vi "HI-POT_Driver.vi"(0 "VISA resource name":refnum<visa-resource-name>, 1 "?":T1, 5 "error in (no error)":errorcluster, 6 "configuration file path":path) -> (9 "Measured Voltage":string, 10 "INTERLOCK STATUS":bool, 11 "Error":bool, 12 "Current":string, 13 "Voltage":string, 14 "VISA resource name out":refnum<visa-resource-name>, 15 "Result":string, 16 "LO SET":string, 17 "Result":bool, 18 "HI SET":string, 19 "error out":errorcluster)   [LabVIEW 2021]
uses:
  Hi-pot_Driver.ctl
  GPT-9800_GSB_L8.5/GPT-9000.lvlib
panel:
  out "substring":string
  out "concatenated string":string
  out "Test Time(S)":dbl
  out "VISA resource name out 4":refnum<visa-resource-name>
  out "VISA resource name out 3":refnum<visa-resource-name>
  out "VISA resource name out 2":refnum<visa-resource-name>
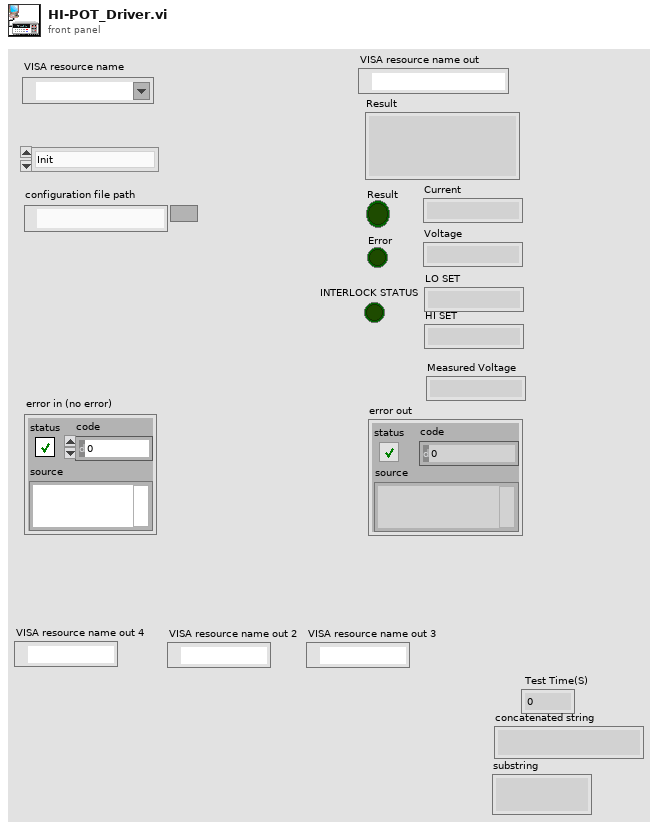
[diagram p1: front panel]
types:
  T1 = typedef "Hi-pot_Driver.ctl" = enum16{"Init ", "Interlock status", "Set UP DCW", "Set UP ACW", "Set UP IR", "Read", "Clear", "Close"}
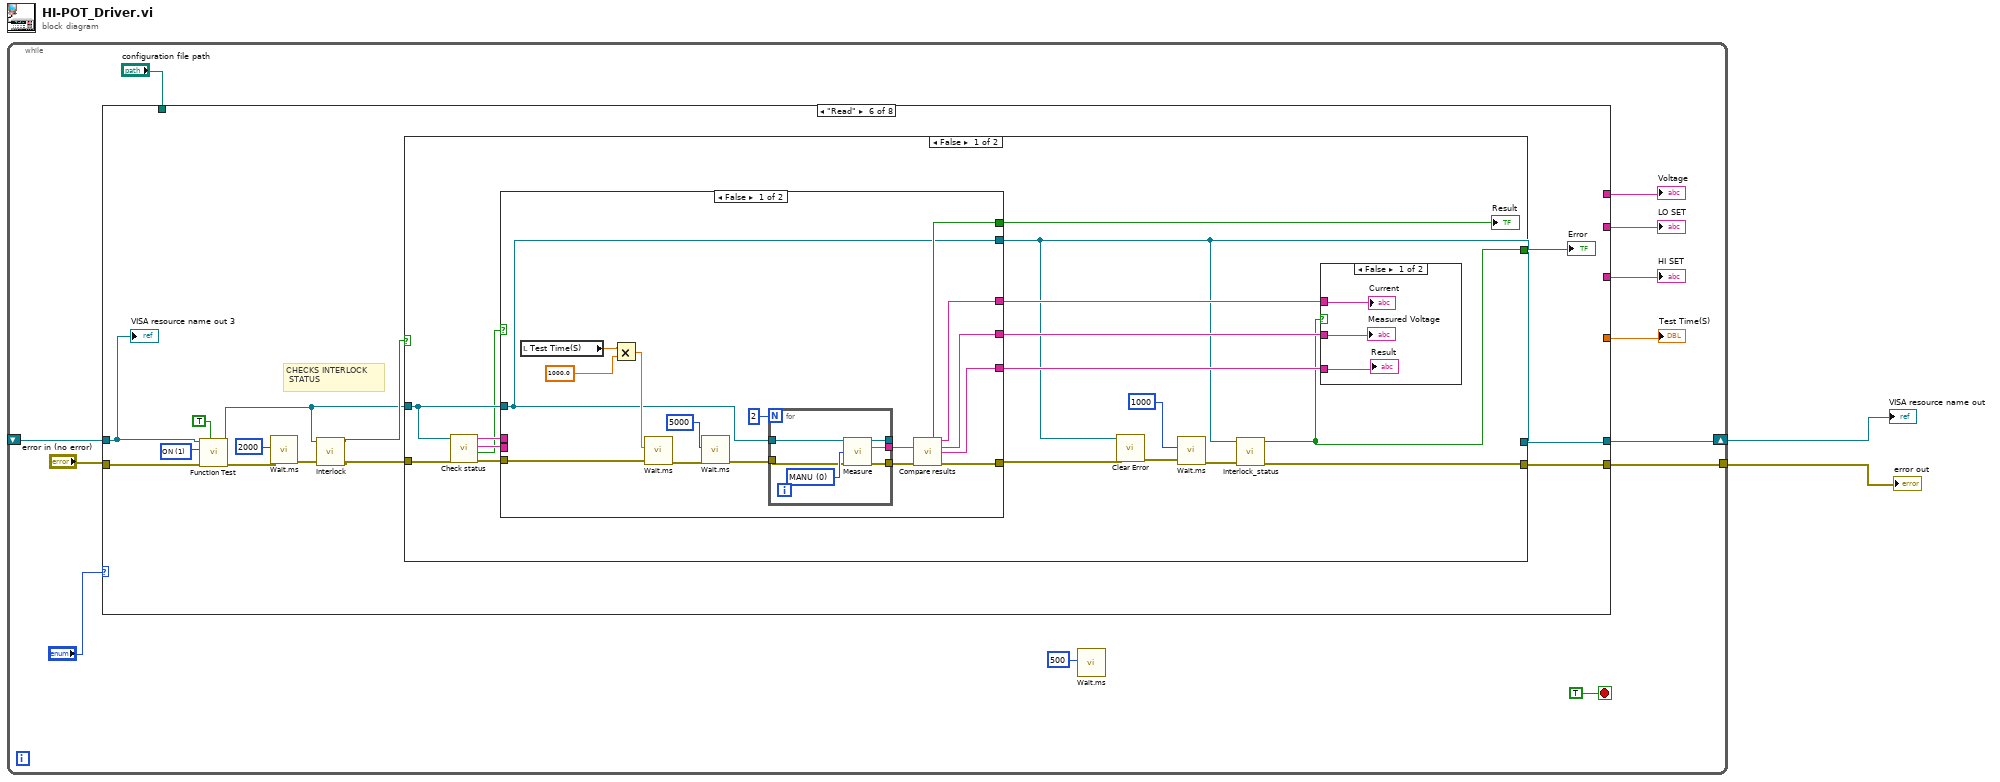
[diagram p0: block diagram]
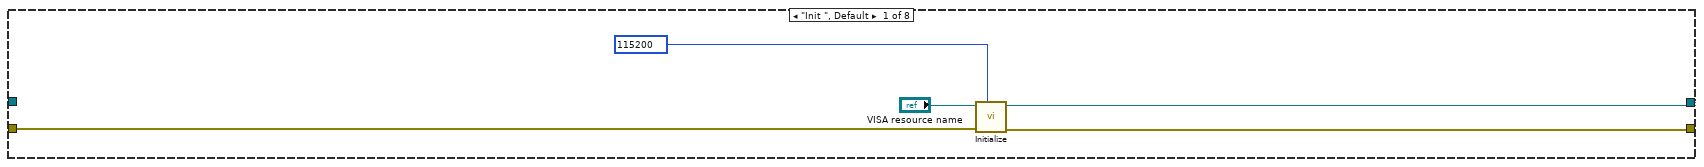
[diagram p2: hidden frame]
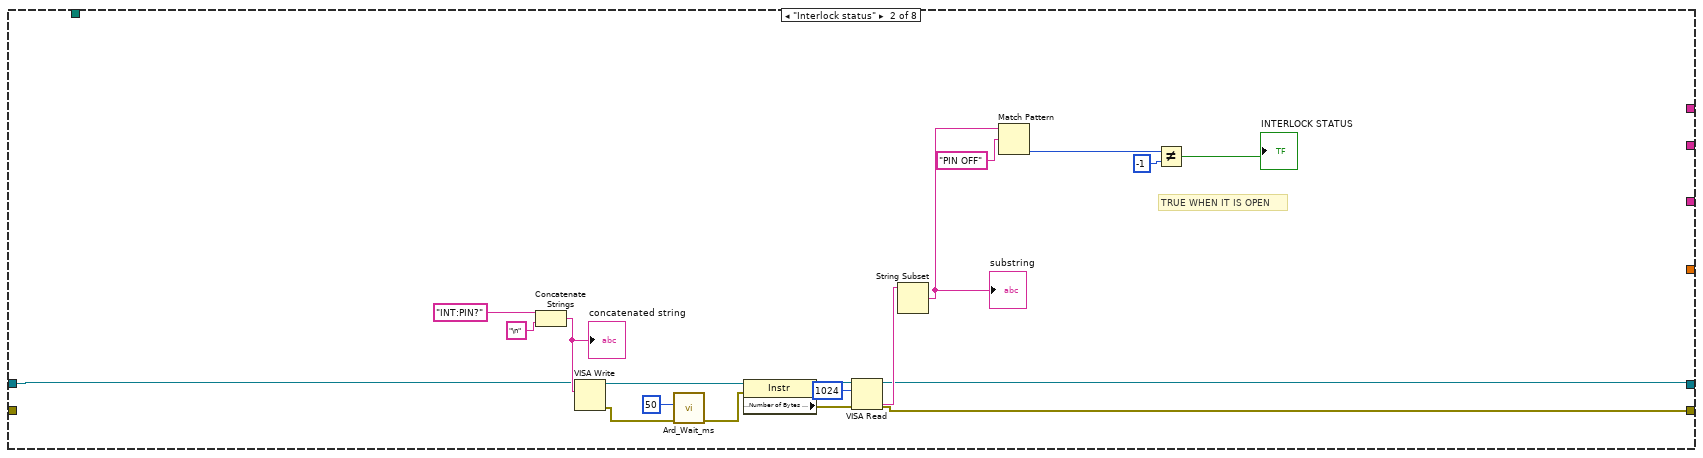
[diagram p3: hidden frame]
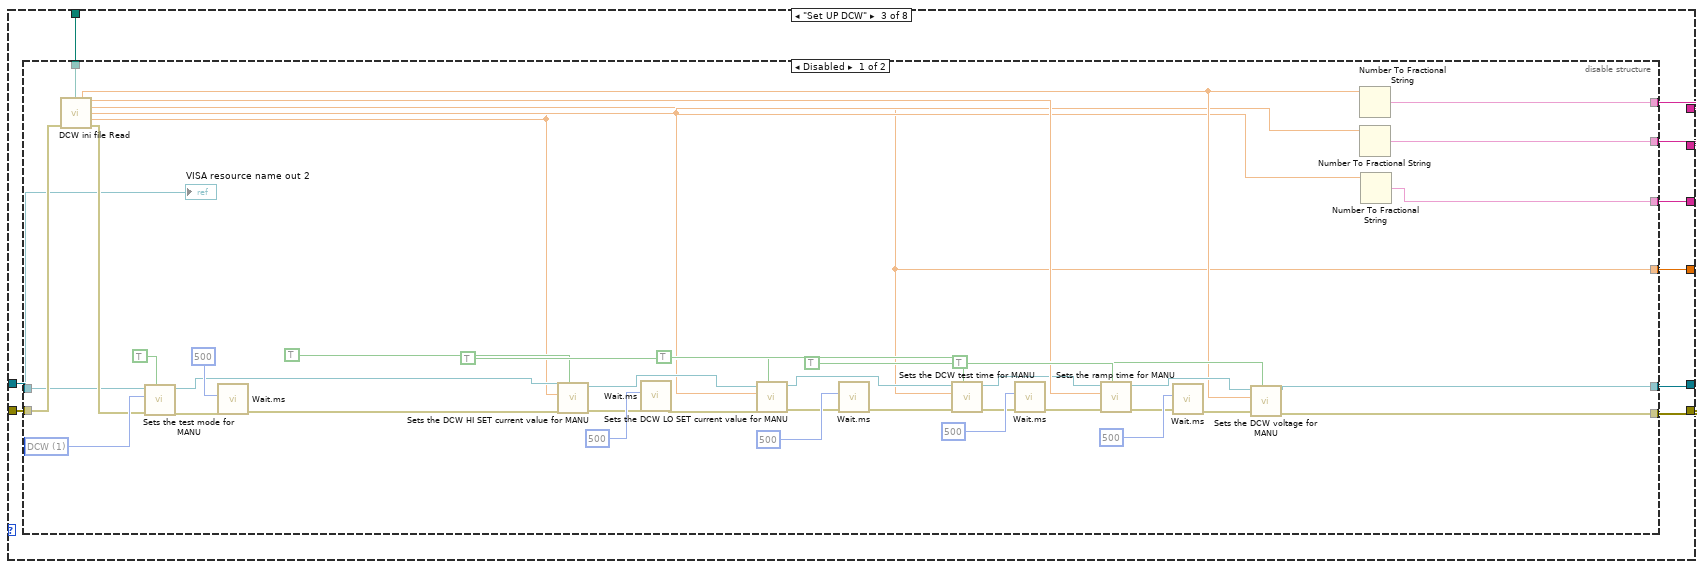
[diagram p4: hidden frame]
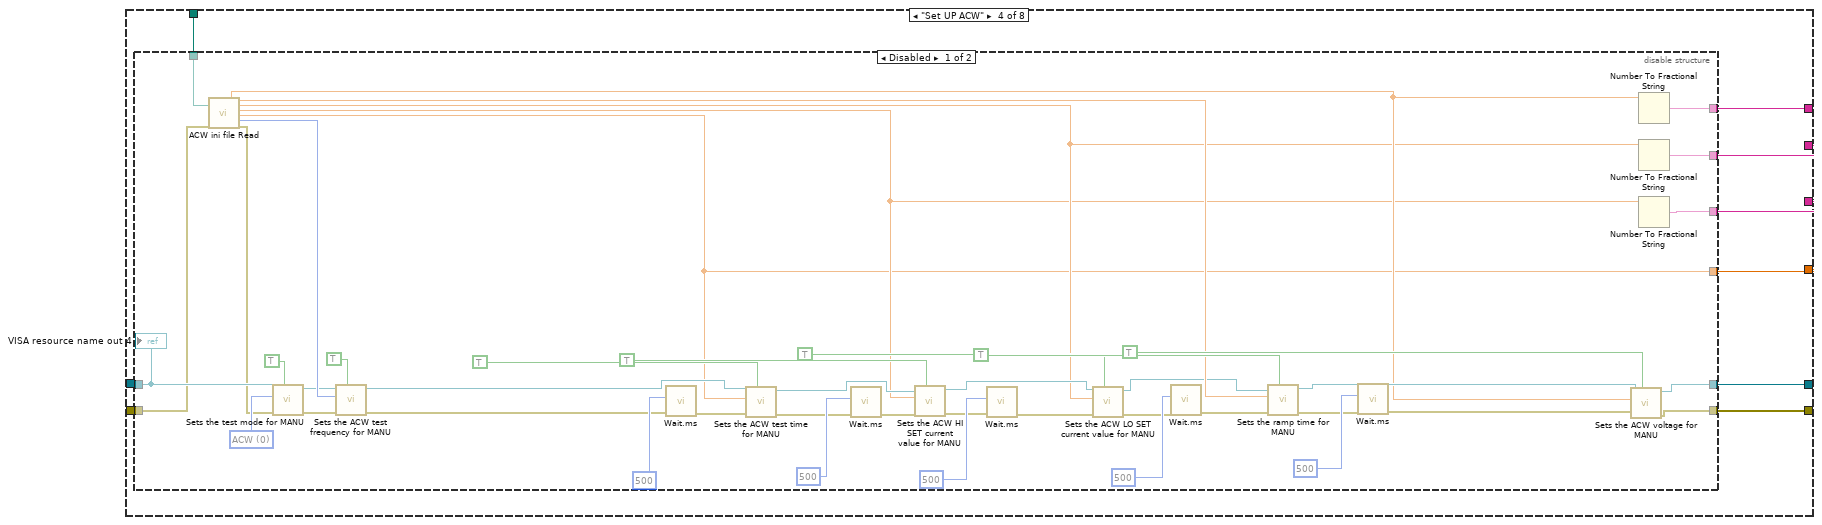
[diagram p6: hidden frame]
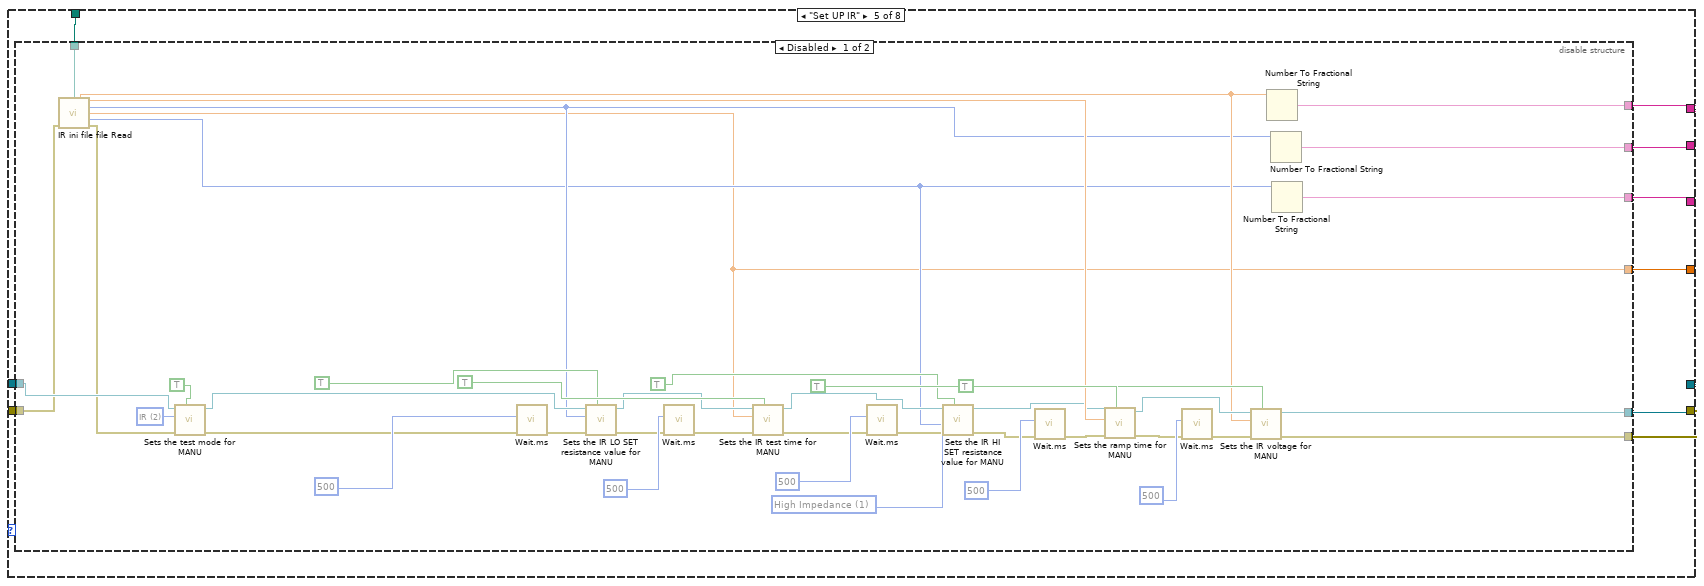
[diagram p8: hidden frame]
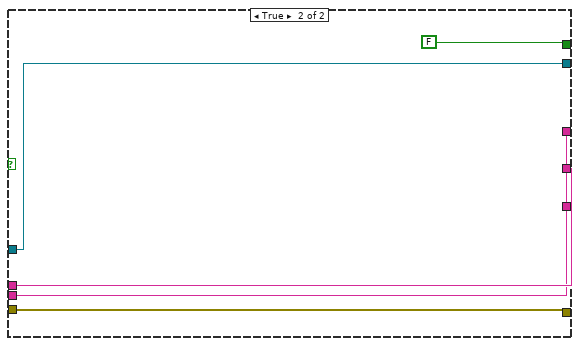
[diagram p11: hidden frame]
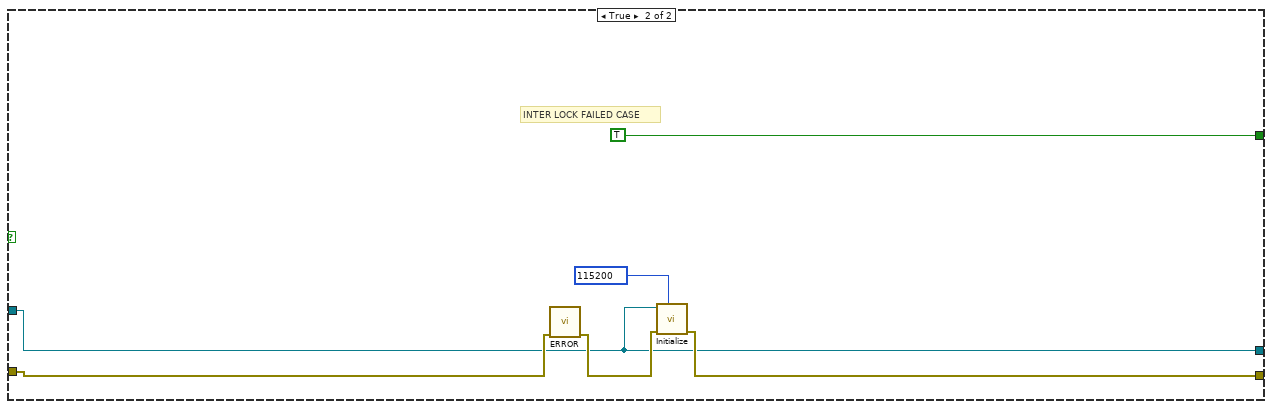
[diagram p12: hidden frame]
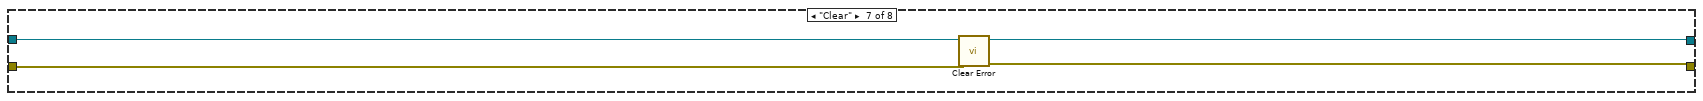
[diagram p13: hidden frame]
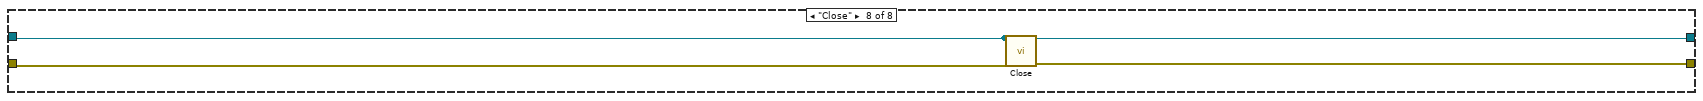
[diagram p14: hidden frame]
diagram:
  n1 = while {
    tunnel: [w3] -> w1
    shift-right: [w13] -> w2
    shift-left: _ -> [w12]
    stop <- TRUE stop-if-true
    n2 = case shown="\"Read\"" "?" {
      tunnel: [w19 w20 w47 w96 w150 w202 w262 w265] -> w3
      tunnel: "error in (no error)" -> [w18 _ w45 w93 w144 w206 w263 w266]
      tunnel: [w16 w21 w39 w95 w149 w201 w260 w264] -> w13
      tunnel: w12 -> [_ w27 w44 w97 w151 w203 w261 w264]
      tunnel: "configuration file path" -> [_ _ w46 w94 w148 _ _ _]
      tunnel: [_ _ w43 w92 w147 _ _ _] -> w8
      tunnel: [_ _ w42 w90 w145 _ _ _] -> w7
      tunnel: [_ _ w41 w91 w146 _ _ _] -> w6
      tunnel: [_ _ w40 w89 w143 _ _ _] -> w5
      frame "Init ", Default {
        w15 = u32 115200 items=["9600"=9600, "19200"=19200, "38400"=38400, "57600"=57600, "115200"=115200] ("Configure RS232 Baud Rate")
        n3 = call "Initialize.vi"("Configure RS232 Baud Rate"=w15, "error in (no error)"=w18, "VISA resource name"="VISA resource name") -> ("error out"=w19:errorcluster, "VISA resource name out"=w16:refnum<visa-resource-name>)  [unwired: 5 in, 2 out]
      }
      frame "Interlock status" {
        # "TRUE WHEN IT IS OPEN"
        n4 = Concatenate Strings("INT:PIN?", "\n" ("string")) -> (w35:string)
        "concatenated string" <- w35
        n5 = VISA Write(VISA resource name=w27, write buffer=w35) -> (VISA resource name out=w36:refnum<visa-resource-name>, error out=w33:errorcluster)  [unwired: 1 in, 1 out]
        n6 = call "Ard_Wait_ms.vi"("error in"=w33, "millisec"=u32 50) -> ("error in 2"=w32:errorcluster)  [unwired: 9 in]
        n7 = property class="Instr" props=["Serial Settings:Number of Bytes at Serial Port"](reference=w36, error in=w32) -> (reference out=w37:refnum<visa-resource-name>, error out=w38:errorcluster)  [unwired: 1 out]
        n8 = VISA Read(VISA resource name=w37, byte count=u32 1024, error in (no error)=w38) -> (VISA resource name out=w21:refnum<visa-resource-name>, read buffer=w30:string, error out=w20:errorcluster)  [unwired: 1 out]
        n9 = String Subset(string=w30) -> (substring=w22:string)  [unwired: 2 in]
        "substring" <- w22
        n10 = Match Pattern(string=w22, regular expression="PIN OFF") -> (offset past match=w24:i32)  [unwired: 1 in, 3 out]
        n11 = Not Equal?(x=w24, y=-1) -> (x != y?=→"INTERLOCK STATUS":bool)
      }
      frame "Set UP DCW" {
        n12 = disable-structure shown="Disabled" {
          disable-tunnel: [w74 _] -> w47
          disable-tunnel: w46 -> [w73 _]
          disable-tunnel: w45 -> [w58 _]
          disable-tunnel: w44 -> [w56 _]
          disable-tunnel: [w54 _] -> w43
          disable-tunnel: [w51 _] -> w42
          disable-tunnel: [w50 _] -> w41
          disable-tunnel: [w49 _] -> w40
          disable-tunnel: [w48 _] -> w39
          frame Disabled {
            w87 = u8 1 items=["ACW", "DCW", "IR", "GB"] ("Test Mode")
            n13 = call "DCW ini file Read.vi"("configuration file path"=w73, "error in (no error) 2"=w58) -> ("DWC Voltage"=w55:dbl, "Ramp Time"=w72:dbl, "DCW Test Time(S)"=w49:dbl, "DCW LO SET"=w53:dbl, "DCW HI SET"=w52:dbl, "error in (no error) 3"=w57:errorcluster)  [unwired: 8 in]
            n14 = call "Sets the test mode for MANU.vi"("Enable to Setup"=TRUE, "error in"=w57, "Test Mode"=w87, "VISA resource name"=w56) -> ("error out"=w85:errorcluster, "VISA resource name out"=w59:refnum<visa-resource-name>)  [unwired: 5 in, 1 out]
            n15 = call "Wait.ms.vi"("error in"=w85, "milliseconds to wait"=u32 500) -> ("error out"=w60:errorcluster)  [unwired: 9 in]
            n16 = call "Sets the DCW HI SET current value for MANU.vi"("Enable to Setup"=TRUE, "error in"=w60, "DCW HI SET current value(mA)"=w52, "VISA resource name"=w59) -> ("error out"=w62:errorcluster, "VISA resource name out"=w61:refnum<visa-resource-name>)  [unwired: 5 in, 1 out]
            n17 = call "Wait.ms.vi"("error in"=w62, "milliseconds to wait"=u32 500) -> ("error out"=w63:errorcluster)  [unwired: 9 in]
            n18 = call "Sets the DCW LO SET current value for MANU.vi"("Enable to Setup"=TRUE, "error in"=w63, "DCW LO SET current value(mA)"=w53, "VISA resource name"=w61) -> ("error out"=w65:errorcluster, "VISA resource name out"=w64:refnum<visa-resource-name>)  [unwired: 5 in, 1 out]
            n19 = call "Wait.ms.vi"("error in"=w65, "milliseconds to wait"=u32 500) -> ("error out"=w66:errorcluster)  [unwired: 9 in]
            n20 = call "Sets the DCW test time for MANU.vi"("Enable to Setup"=TRUE, "error in"=w66, "DCW Test Time(S)"=w49, "VISA resource name"=w64) -> ("error out"=w67:errorcluster, "VISA resource name out"=w68:refnum<visa-resource-name>)  [unwired: 5 in, 1 out]
            n21 = call "Wait.ms.vi"("error in"=w67, "milliseconds to wait"=u32 500) -> ("error out"=w69:errorcluster)  [unwired: 9 in]
            n22 = call "Sets the ramp time for MANU.vi"("Enable to Setup"=TRUE, "error in"=w69, "Ramp Time"=w72, "VISA resource name"=w68) -> ("error out"=w71:errorcluster, "VISA resource name out"=w70:refnum<visa-resource-name>)  [unwired: 5 in, 1 out]
            n23 = call "Wait.ms.vi"("error in"=w71, "milliseconds to wait"=u32 500) -> ("error out"=w75:errorcluster)  [unwired: 9 in]
            n24 = call "Sets the DCW voltage for MANU.vi"("Enable to Setup"=TRUE, "error in"=w75, "DCW voltage(kV)"=w55, "VISA resource name"=w70) -> ("error out"=w74:errorcluster, "VISA resource name out"=w48:refnum<visa-resource-name>)  [unwired: 5 in, 1 out]
            n25 = Number To Fractional String(number=w55) -> (F-format string=w54:string)  [unwired: 3 in]
            n26 = Number To Fractional String(number=w53) -> (F-format string=w51:string)  [unwired: 3 in]
            n27 = Number To Fractional String(number=w52) -> (F-format string=w50:string)  [unwired: 3 in]
            "VISA resource name out 2" <- w56
          }
          frame Enabled {
          }
        }
      }
      frame "Set UP ACW" {
        n28 = disable-structure shown="Disabled" {
          disable-tunnel: w97 -> [w141 _]
          disable-tunnel: [w133 _] -> w96
          disable-tunnel: [w132 _] -> w95
          disable-tunnel: w94 -> [w127 _]
          disable-tunnel: w93 -> [w107 _]
          disable-tunnel: [w104 _] -> w92
          disable-tunnel: [w103 _] -> w91
          disable-tunnel: [w99 _] -> w90
          disable-tunnel: [w98 _] -> w89
          frame Disabled {
            w140 = u8 0 items=["ACW", "DCW", "IR", "GB"] ("Test Mode")
            n29 = call "ACW ini file Read.vi"("error in (no error) 2"=w107, "configuration file path"=w127) -> ("ACW Voltage"=w105:dbl, "Ramp Time"=w123:dbl, "LO SET"=w102:dbl, "HI SET"=w101:dbl, "Test Time"=w98:dbl, "Freq"=w112:u32, "error in (no error) 3"=w106:errorcluster)  [unwired: 11 in]
            n30 = call "Sets the test mode for MANU.vi"("Enable to Setup"=TRUE, "error in"=w106, "Test Mode"=w140, "VISA resource name"=w141) -> ("error out"=w109:errorcluster, "VISA resource name out"=w108:refnum<visa-resource-name>)  [unwired: 5 in, 1 out]
            n31 = call "Sets the ACW test frequency for MANU.vi"("Enable to Setup"=TRUE, "error in"=w109, "ACW Test Frequency(Hz)"=w112, "VISA resource name"=w108) -> ("error out"=w110:errorcluster, "VISA resource name out"=w100:refnum<visa-resource-name>)  [unwired: 5 in, 1 out]
            n32 = call "Wait.ms.vi"("error in"=w110, "milliseconds to wait"=u32 500) -> ("error out"=w111:errorcluster)  [unwired: 9 in]
            n33 = call "Sets the ACW test time for MANU.vi"("Enable to Setup"=TRUE, "error in"=w111, "ACW Test Time(S)"=w98, "VISA resource name"=w100) -> ("error out"=w115:errorcluster, "VISA resource name out"=w114:refnum<visa-resource-name>)  [unwired: 5 in, 1 out]
            n34 = call "Wait.ms.vi"("error in"=w115, "milliseconds to wait"=u32 500) -> ("error out"=w116:errorcluster)  [unwired: 9 in]
            n35 = call "Sets the ACW HI SET current value for MANU.vi"("Enable to Setup"=TRUE, "error in"=w116, "ACW HI SET current value(mA)"=w101, "VISA resource name"=w114) -> ("error out"=w117:errorcluster, "VISA resource name out"=w113:refnum<visa-resource-name>)  [unwired: 5 in, 1 out]
            n36 = call "Wait.ms.vi"("error in"=w117, "milliseconds to wait"=u32 500) -> ("error out"=w118:errorcluster)  [unwired: 9 in]
            n37 = call "Sets the ACW LO SET current value for MANU.vi"("Enable to Setup"=TRUE, "error in"=w118, "ACW LO SET current value(mA)"=w102, "VISA resource name"=w113) -> ("error out"=w121:errorcluster, "VISA resource name out"=w120:refnum<visa-resource-name>)  [unwired: 5 in, 1 out]
            n38 = call "Wait.ms.vi"("error in"=w121, "milliseconds to wait"=u32 500) -> ("error out"=w122:errorcluster)  [unwired: 9 in]
            n39 = call "Sets the ramp time for MANU.vi"("Enable to Setup"=TRUE, "error in"=w122, "Ramp Time"=w123, "VISA resource name"=w120) -> ("error out"=w124:errorcluster, "VISA resource name out"=w119:refnum<visa-resource-name>)  [unwired: 5 in, 1 out]
            n40 = call "Wait.ms.vi"("error in"=w124, "milliseconds to wait"=u32 500) -> ("error out"=w125:errorcluster)  [unwired: 9 in]
            n41 = call "Sets the ACW voltage for MANU.vi"("Enable to Setup"=TRUE, "error in"=w125, "ACW voltage(kV)"=w105, "VISA resource name"=w119) -> ("error out"=w133:errorcluster, "VISA resource name out"=w132:refnum<visa-resource-name>)  [unwired: 5 in, 1 out]
            n42 = Number To Fractional String(number=w105) -> (F-format string=w104:string)  [unwired: 3 in]
            n43 = Number To Fractional String(number=w102) -> (F-format string=w99:string)  [unwired: 3 in]
            n44 = Number To Fractional String(number=w101) -> (F-format string=w103:string)  [unwired: 3 in]
            "VISA resource name out 4" <- w141
          }
          frame Enabled {
          }
        }
      }
      frame "Set UP IR" {
        n45 = disable-structure shown="Disabled" {
          disable-tunnel: w151 -> [w192 _]
          disable-tunnel: [w183 _] -> w150
          disable-tunnel: [w182 _] -> w149
          disable-tunnel: w148 -> [w176 _]
          disable-tunnel: [w160 _] -> w147
          disable-tunnel: [w158 _] -> w146
          disable-tunnel: [w157 _] -> w145
          disable-tunnel: w144 -> [w156 _]
          disable-tunnel: [w152 _] -> w143
          frame Disabled {
            w177 = u8 1 items=["High Impedance"=1, "Setup as below"=0] ("Sets value to high impedance")
            w191 = u8 2 items=["ACW", "DCW", "IR", "GB"] ("Test Mode")
            n46 = call "IR ini file file Read.vi"("configuration file path"=w176, "error in (no error) 2"=w156) -> ("IR Voltage"=w159:dbl, "Ramp Time"=w172:dbl, "IR LO SET resistance value(M£[)"=w154:u16, "IR Time"=w152:dbl, "IR HI SET resistance value(M£[)"=w153:u16, "error in (no error) 3"=w155:errorcluster)  [unwired: 8 in]
            n47 = call "Sets the test mode for MANU.vi"("Enable to Setup"=TRUE, "error in"=w155, "Test Mode"=w191, "VISA resource name"=w192) -> ("error out"=w189:errorcluster, "VISA resource name out"=w162:refnum<visa-resource-name>)  [unwired: 5 in, 1 out]
            n48 = call "Wait.ms.vi"("error in"=w189, "milliseconds to wait"=u32 500) -> ("error out"=w163:errorcluster)  [unwired: 9 in]
            n49 = call "Sets the IR LO SET resistance value for MANU.vi"("Enable to Setup"=TRUE, "error in"=w163, "IR LO SET resistance value(M£[)"=w154, "VISA resource name"=w162) -> ("error out"=w164:errorcluster, "VISA resource name out"=w161:refnum<visa-resource-name>)  [unwired: 5 in, 1 out]
            n50 = call "Wait.ms.vi"("error in"=w164, "milliseconds to wait"=u32 500) -> ("error out"=w165:errorcluster)  [unwired: 9 in]
            n51 = call "Sets the IR test time for MANU.vi"("Enable to Setup"=TRUE, "error in"=w165, "IR Test Time(S)"=w152, "VISA resource name"=w161) -> ("error out"=w167:errorcluster, "VISA resource name out"=w166:refnum<visa-resource-name>)  [unwired: 5 in, 1 out]
            n52 = call "Wait.ms.vi"("error in"=w167, "milliseconds to wait"=u32 500) -> ("error out"=w168:errorcluster)  [unwired: 9 in]
            n53 = call "Sets the IR HI SET resistance value for MANU.vi"("Enable to Setup"=TRUE, "error in"=w168, "IR HI SET resistance value(M£[)"=w153, "Sets value to high impedance"=w177, "VISA resource name"=w166) -> ("error out"=w170:errorcluster, "VISA resource name out"=w169:refnum<visa-resource-name>)  [unwired: 4 in, 1 out]
            n54 = call "Wait.ms.vi"("error in"=w170, "milliseconds to wait"=u32 500) -> ("error out"=w171:errorcluster)  [unwired: 9 in]
            n55 = call "Sets the ramp time for MANU.vi"("Enable to Setup"=TRUE, "error in"=w171, "Ramp Time"=w172, "VISA resource name"=w169) -> ("error out"=w173:errorcluster, "VISA resource name out"=w174:refnum<visa-resource-name>)  [unwired: 5 in, 1 out]
            n56 = call "Wait.ms.vi"("error in"=w173, "milliseconds to wait"=u32 500) -> ("error out"=w175:errorcluster)  [unwired: 9 in]
            n57 = call "Sets the IR voltage for MANU.vi"("Enable to Setup"=TRUE, "error in"=w175, "IR voltage(kV)"=w159, "VISA resource name"=w174) -> ("error out"=w183:errorcluster, "VISA resource name out"=w182:refnum<visa-resource-name>)  [unwired: 5 in, 1 out]
            n58 = Number To Fractional String(number=w159) -> (F-format string=w160:string)  [unwired: 3 in]
            n59 = Number To Fractional String(number=w154) -> (F-format string=w157:string)  [unwired: 3 in]
            n60 = Number To Fractional String(number=w153) -> (F-format string=w158:string)  [unwired: 3 in]
          }
          frame Enabled {
          }
        }
      }
      frame "Read" {
        w204 = u8 1 items=["OFF", "ON"] ("Function Test")
        # "CHECKS INTERLOCK\n STATUS"
        n61 = call "Function Test.vi"("VISA resource name"=w203, "Function Test"=w204, "error in"=w206, "Enable to Setup"=TRUE) -> ("VISA resource name out"=w198:refnum<visa-resource-name>, "error out"=w197:errorcluster)  [unwired: 4 in, 1 out]
        n62 = call "Wait.ms.vi"("error in"=w197, "milliseconds to wait"=u32 2000) -> ("error out"=w196:errorcluster)  [unwired: 9 in]
        n63 = call "Interlock.vi"("error in"=w196, "VISA resource name"=w198) -> ("error out"=w200:errorcluster, "RESULT"=w199:bool)  [unwired: 8 in]
        n64 = case shown="False" w199 {
          tunnel: w198 -> [w221 w256]
          tunnel: [w217 w257] -> w202
          tunnel: [w211 w256] -> w201
          tunnel: w200 -> [w222 w259]
          tunnel: [w207 TRUE] -> w194
          frame False {
            n65 = call "Check status.vi"("error in"=w222, "VISA resource name"=w221) -> ("error out"=w223:errorcluster, "RESULT"=w218:bool, "Current"=w219:string, "Voltage"=w220:string)  [unwired: 6 in]
            n66 = case shown="False" w218 {
              tunnel: [w238 FALSE] -> w208
              tunnel: [w237 w251] -> w215
              tunnel: [w236 w252] -> w214
              tunnel: w223 -> [w239 w249]
              tunnel: w221 -> [w228 w250]
              tunnel: w220 -> [_ w252]
              tunnel: w219 -> [_ w251]
              tunnel: [w235 _] -> w213
              tunnel: [w228 w250] -> w211
              tunnel: [w227 w249] -> w210
              frame False {
                n67 = local read "Test Time(S)"() -> (w242:dbl)
                n68 = Multiply(x=w242, y=1000.0) -> (x*y=w240:dbl)
                n69 = call "Wait.ms.vi"("error in"=w239, "milliseconds to wait"=w240) -> ("error out"=w234:errorcluster)  [unwired: 9 in]
                n70 = call "Wait.ms.vi"("error in"=w234, "milliseconds to wait"=u32 5000) -> ("error out"=w229:errorcluster)  [unwired: 9 in]
                n71 = for {
                  N: 2 -> [_]
                  tunnel: [w247] -> w231
                  tunnel: [w245] -> w232
                  tunnel: w228 -> [w246]
                  tunnel: [w244] -> _
                  tunnel: w229 -> [w243]
                  w248 = u8 0 items=["MANU", "AUTO"] ("Function Mode Numeric")
                  n72 = call "Measure.vi"("VISA resource name"=w246, "Function Mode Numeric"=w248, "error in"=w243) -> ("VISA resource name out"=w244:refnum<visa-resource-name>, "Return  the test status"=w247:string, "error out"=w245:errorcluster)  [unwired: 9 in, 1 out]
                }
                n73 = call "Compare results.vi"("string"=w231, 11:w232) -> (3:"Result"=w238:bool, "Current"=w237:string, "Measured Voltage"=w236:string, 8:"Result"=w235:string, 15:w227:errorcluster)  [unwired: 9 in]
              }
              frame True {
              }
            }
            "Result" <- w208
            n74 = call "Clear Error.vi"("error in (no error)"=w210, "VISA resource name"=w211) -> ("error out"=w212:errorcluster)  [unwired: 8 in, 1 out]
            n75 = call "Wait.ms.vi"("error in"=w212, "milliseconds to wait"=u32 1000) -> ("error out"=w209:errorcluster)  [unwired: 9 in]
            n76 = call "Interlock_status.vi"("error in (no error)"=w209, "VISA resource name"=w211) -> ("error out"=w217:errorcluster, "INTERLOCK STATUS"=w207:bool)  [unwired: 8 in]
            n77 = case shown="False" w207 {
              tunnel: w215 -> [w226 _]
              tunnel: w214 -> [w225 _]
              tunnel: w213 -> [w224 _]
              frame False {
                "Current" <- w226
                "Measured Voltage" <- w225
                "Result" <- w224
              }
              frame True {
              }
            }
          }
          frame True {
            w255 = u32 115200 items=["9600"=9600, "19200"=19200, "38400"=38400, "57600"=57600, "115200"=115200] ("Configure RS232 Baud Rate")
            # "INTER LOCK FAILED CASE"
            n78 = call "ERROR.vi"(8:w259) -> ("error"=w258:errorcluster)  [unwired: 10 in]
            n79 = call "Initialize.vi"("Configure RS232 Baud Rate"=w255, "error in (no error)"=w258, "VISA resource name"=w256) -> ("error out"=w257:errorcluster)  [unwired: 5 in, 3 out]
          }
        }
        "Error" <- w194
        "VISA resource name out 3" <- w203
      }
      frame "Clear" {
        n80 = call "Clear Error.vi"("error in (no error)"=w263, "VISA resource name"=w261) -> ("error out"=w262:errorcluster, "VISA resource name out"=w260:refnum<visa-resource-name>)  [unwired: 8 in]
      }
      frame "Close" {
        n81 = call "Close.vi"("error in (no error)"=w266, "VISA resource name"=w264) -> ("error out"=w265:errorcluster)  [unwired: 9 in]
      }
    }
    "Voltage" <- w8
    "LO SET" <- w7
    "HI SET" <- w6
    "Test Time(S)" <- w5
    n82 = call "Wait.ms.vi"("milliseconds to wait"=u32 500) -> ()  [unwired: 10 in, 1 out]
  }
  "error out" <- w1
  "VISA resource name out" <- w2
